vi "Add Fixture Two Questions Tool.vi"(8 "error in (no error)":errorcluster, 11 "server id":i32) -> (0 "error out":errorcluster, 3 "server id out":i32)   [LabVIEW 2020, in "MCP Server tests.lvlib"]
doc: "Test helper. Registers fake tool two questions.vi, which lies beside this VI, as an MCP tool."
uses:
  MCP Server tests.lvlib
  src/MCP Server/MCP Server.lvlib
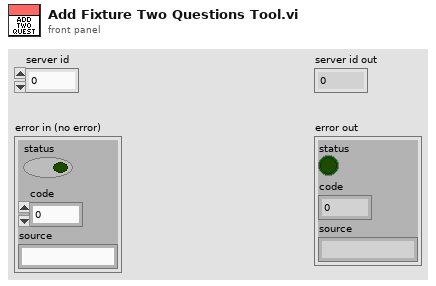
[diagram p1: front panel]
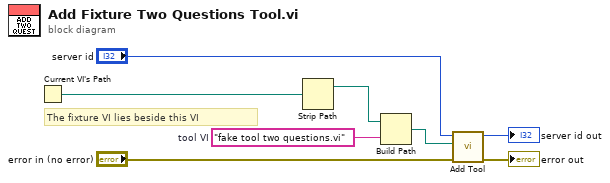
[diagram p0: block diagram]
diagram:
  w3 = "fake tool two questions.vi"  # tool VI
  # "The fixture VI lies beside this VI"
  n1 = Current VI's Path() -> (path=w4:path)
  n2 = Strip Path(path=w4) -> (stripped path=w5:path)  [unwired: 1 out]
  n3 = Build Path(base path=w5, name or relative path=w3) -> (appended path=w6:path)
  n4 = call "Add Tool.vi"("error in (no error)"="error in (no error)", "vi path"=w6, "server id"="server id") -> ("error out"=→"error out":errorcluster, "server id out"=→"server id out":i32)  [unwired: 7 in]
